vi "[ce] ODE - VM Error Handler.vi"(5 "var name":string, 6 "error before":errorcluster, 9 "err code":T1 items=["No error", "Invalid variable type", "Variable not found", "Variable already exists", "Invalid context handle", "Input error", "Invalid data format", "No history attached", "History already attached", "Invalid history parameters", "Wrong variable name", "Wrong alias name", "Non-unique alias", "Alias not found", "No alias associated", "Alias already associated", "Wrong context name", "Non-unique context name", "Context name not found", "Invalid parameter", "Generic error", "Memory Full", "Unrecognized LV error", "Unknown error code"]) -> (0 "error out":errorcluster)   [LabVIEW 2021]
doc: "::: CalcExpress Toolkit :::\nCopyright (c) 2000-2026 Konstantin Shifershteyn. All rights reserved."
uses:
  cetypes.llb/VarMan Error Code.ctl
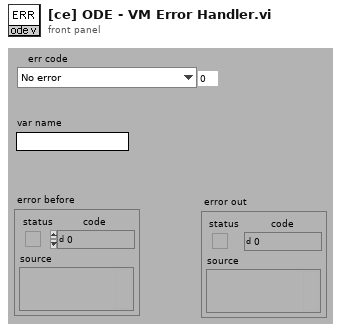
[diagram p1: front panel]
types:
  T1 = typedef "VarMan Error Code.ctl" = u16
  T2 = enum16{"ok", "invalid type", "var not def", "var already def", "inv handle", "input error", "invalid data format", "unknown error"}
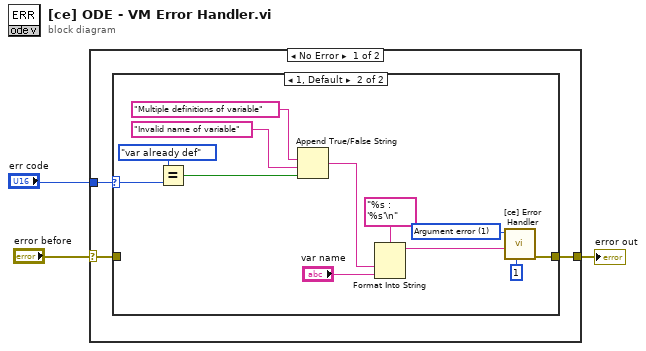
[diagram p0: block diagram]
diagram:
  n1 = case shown="No Error" "error before" {
    selector: "error before" -> [w4 w20]
    tunnel: [w6 w20] -> w3
    tunnel: "err code" -> [w5 _]
    frame No Error {
      n2 = case shown="1, Default" w5 {
        selector: w5 -> [_ w18]
        tunnel: [w7 w11] -> w6
        tunnel: w4 -> [w7 _]
        frame 0 {
        }
        frame 1, Default {
          w9 = u16 1 items=["No error", "Argument error", "Memory is full", "Out of zone", "End of file", "File already open", "Generic file I/O error", "File not found", "File permission error", "Disk is full", "Duplicate path", "Too many files open", "System feature not enabled", "Resource file not found", "Cannot add resource", "Resource not found", "Image not found", "Image memory error", "Pen does not exist", "Config type invalid", "Config token not found", "Config parse error", "Config memory error", "Bad external code format", "Bad external code offset", "External code not present", "Null window", "Destroy window error", "Null menu", "Print aborted", "Bad print record", "Print driver error", "Windows error during printing", "Memory error during printing", "Print dialog error", "Generic print error", "Invalid device refnum", "Device not found", "Device parameter error", "Device unit error", "Cannot open device", "Device call aborted", "Generic error", "Cancelled by user", "Object ID too low", "Object ID too high", "Object not in heap", "Unknown heap", "Unknown object (invalid DefProc)", "Unknown object (DefProc not in table)", "Message out of range", "Invalid (null) method", "Unknown message", "Manager call not supported", "Bad address", "Network operation in progress", "Network operation timed out", "Connection is busy", "Network attribute not supported", "Network error", "Address in use", "System out of memory", "Connection aborted", "Connection refused", "Not connected", "Already connected", "Connection closed", "Initialization error (interapplication manager)", "Bad occurrence", "Wait on unbound occurrence handler", "Occurrence queue overflow", "Datalog type conflict", "Unused", "Unrecognized type (interapplication manager)", "Memory corrupt", "Failed to make temporary DLL", "Old CIN version", "Drag socket not found", "Failed to load drop-object", "Failed to register OLE object", "Failed to release OLE object", "Format specifier type mismatch", "Unknown format specifier", "Too few format specifiers", "Too many format specifiers", "Scan failed", "Newer CIN version", "OLE Convert", "Runtime menu error", "Password tampered", "Unknown error code"]
          n3 = Equal?(x=T2."var already def" ("err code"), y=w18) -> (x = y?=w16:bool)
          n4 = Append True/False String(1:w16, 2:"Invalid name of variable" ("false string"), 3:"Multiple definitions of variable" ("true string")) -> (0:w13:string)  [unwired: 1 in]
          n5 = Format Into String(format string="%s : '%s'\n", w13, "var name") -> (resulting string=w10:string)  [unwired: 2 in, 1 out]
          n6 = call "[ce] Error Handler.vi"("nesting level"=1, "error reason"=w10, "error code"=w9) -> ("error out"=w11:errorcluster)  [unwired: 7 in, 1 out]
        }
      }
    }
    frame Error {
    }
  }
  "error out" <- w3
